vi "Start Sync.vi"(8 "error in (no error)":errorcluster, 11 "gRPC service in":refnum<class "OOBgRPCService.lvclass">) -> (0 "error out":errorcluster, 3 "gRPC service out":refnum<class "OOBgRPCService.lvclass">)   [LabVIEW 2025, in "OOB gRPC Server.lvlib" / "OOBgRPCService.lvclass"]
uses:
  OOBgRPCService.lvclass
  OOBgRPCService.lvclass/OOBgRPCService.ctl
  RPC Messages/hwval_GenericResponse.ctl
  <vilib>/xnet/xnet.llb/XNET Frame Type CAN.ctl
  RPC Messages/hwval_StatusResponse.ctl
  OOB Data Transfer/OOB Data Transfer.lvlib
  OOB gRPC Server.lvlib
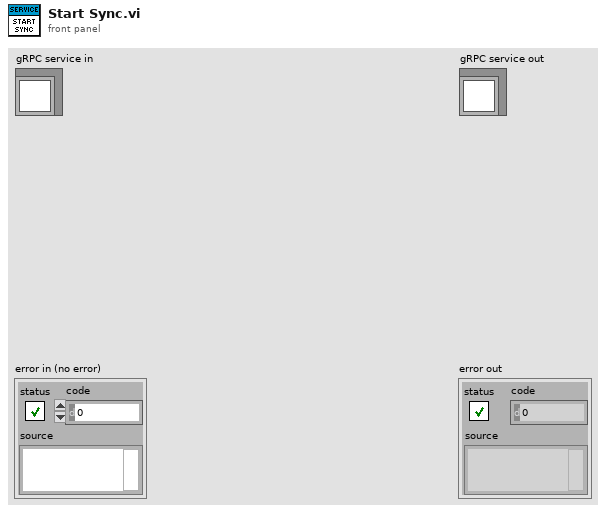
[diagram p1: front panel]
types:
  T1 = typedef "OOB gRPC Server.lvlib/hwval_GenericResponse.ctl" = cluster{"Payload":u8[]}
  T2 = typedef "OOB gRPC Server.lvlib/hwval_StatusResponse.ctl" = cluster{"Status":bool, "Code":i32, "Message":string}
  T3 = typedef "OOB gRPC Server.lvlib/OOBgRPCService.lvclass/Server Internal UEs.ctl" = cluster{"OOBgRPCService Generic Internal UE":refnum<user-event>, "OOBgRPCService PauseResume Internal UE":refnum<user-event>, "OOBgRPCService Export Internal UE":refnum<user-event>}
  T4 = typedef "OOB gRPC Server.lvlib/OOBgRPCService.lvclass/Server gRPC UEs.ctl" = cluster{"OOBgRPCService Generic gRPC UE":refnum<user-event>, "OOBgRPCService PauseResume gRPC UE":refnum<user-event>, "OOBgRPCService Export gRPC UE":refnum<user-event>}
  T5 = typedef "grpc-lvsupport-release.lvlib/grpcId.ctl" = u64
  T6 = typedef "OOB gRPC Server.lvlib/hwval_GenericRequest.ctl" = cluster{"Command":string, "Payload":u8[]}
  T7 = typedef "OOB Data Transfer.lvlib/OOB to Logic Data.ctl" = cluster{"PauseResume":bool, "Export":string, "ID CAN":u32, "Type CAN":T8, "DLC CAN":u32, "SEND CAN":bool, "Payload CAN":u32[], "ID LIN":u32, "DLC LIN":u32, "SEND LIN":bool, "Payload LIN":u32[], "out_str":string, "cfg err":bool}
  T8 = typedef "XNET Frame Type CAN.ctl" = u8
  T9 = typedef "OOB gRPC Server.lvlib/hwval_BoolRequest.ctl" = cluster{"BooleanData":bool}
  T10 = typedef "OOB gRPC Server.lvlib/hwval_ExportRequest.ctl" = cluster{"FileType":string}
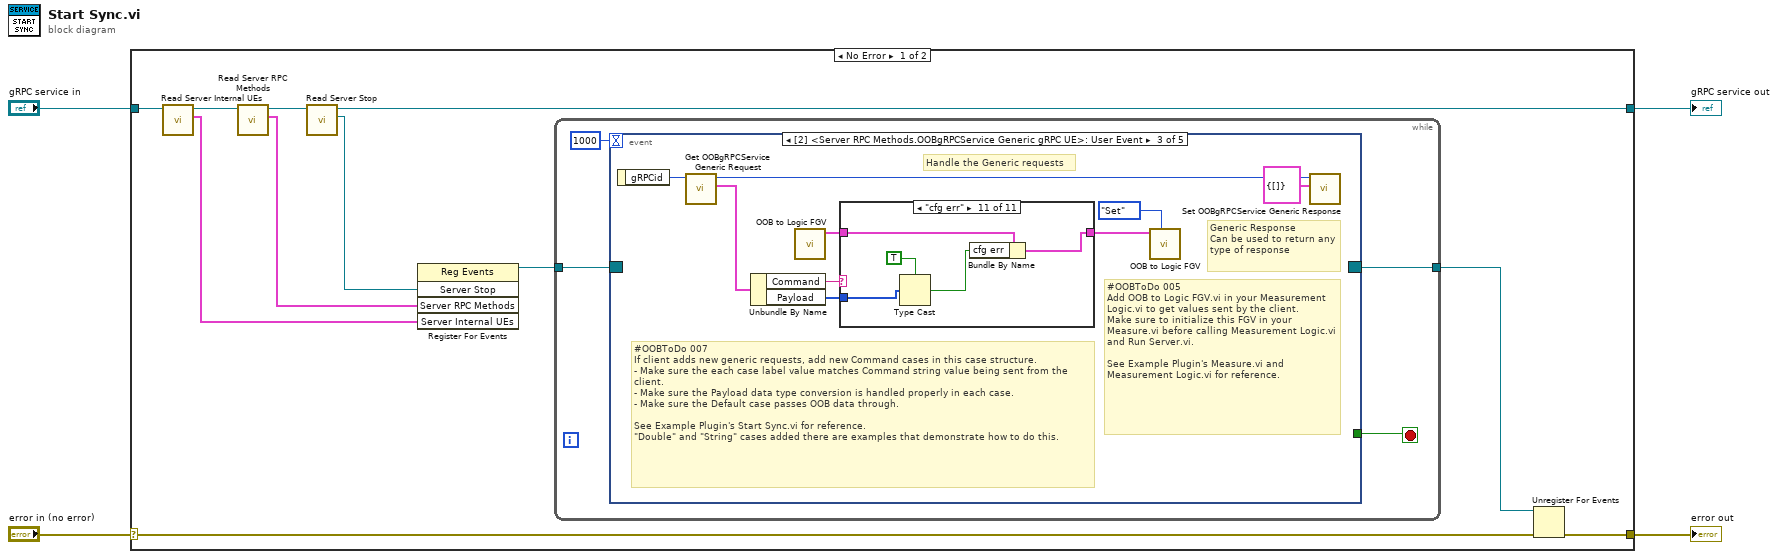
[diagram p0: block diagram]
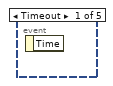
[diagram p2: hidden frame]
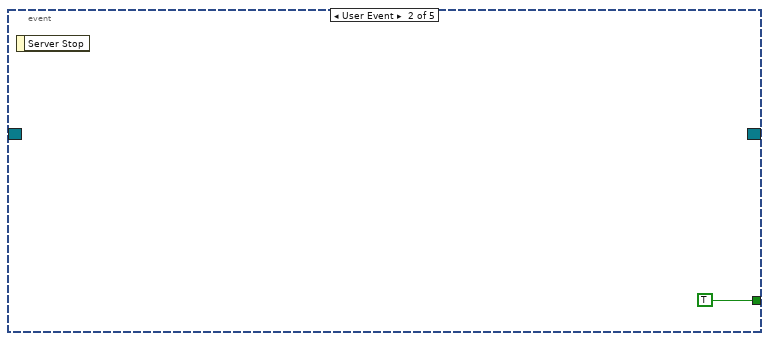
[diagram p3: hidden frame]
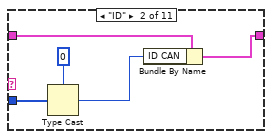
[diagram p5: hidden frame]
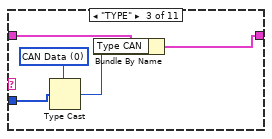
[diagram p6: hidden frame]
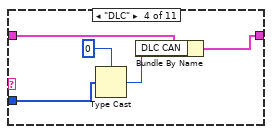
[diagram p7: hidden frame]
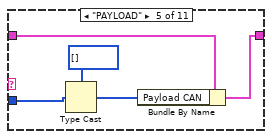
[diagram p8: hidden frame]
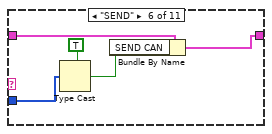
[diagram p9: hidden frame]
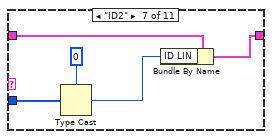
[diagram p10: hidden frame]
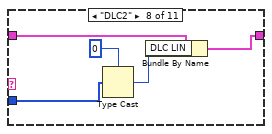
[diagram p11: hidden frame]
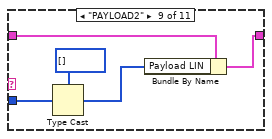
[diagram p12: hidden frame]
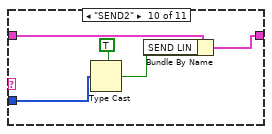
[diagram p13: hidden frame]
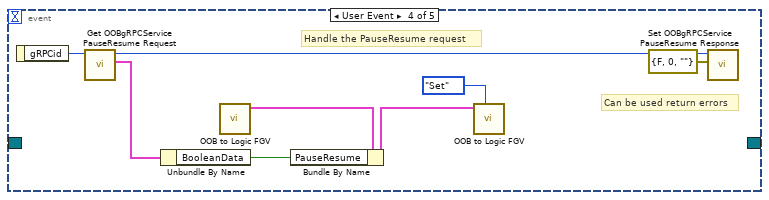
[diagram p14: hidden frame]
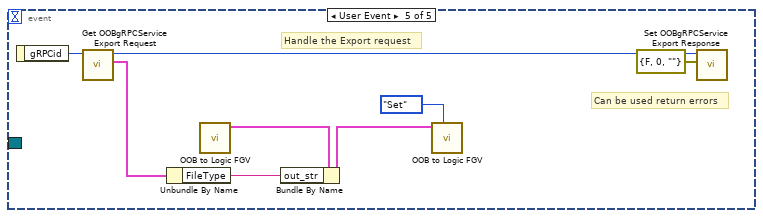
[diagram p15: hidden frame]
diagram:
  n1 = case shown="No Error" "error in (no error)" {
    selector: "error in (no error)" -> [w9 w98]
    tunnel: [w8 w98] -> w3
    tunnel: [w6 w97] -> w1
    tunnel: "gRPC service in" -> [w15 w97]
    frame No Error {
      n2 = call "Read Server Internal UEs.vi"("gRPC service in"=w15) -> ("Server Internal UEs"=w13:T3, "gRPC service out"=w14:refnum<class "OOBgRPCService.lvclass">)  [unwired: 8 in, 1 out]
      n3 = call "Read Server RPC Methods.vi"("gRPC service in"=w14) -> ("Server RPC Methods"=w7:T4, "gRPC service out"=w12:refnum<class "OOBgRPCService.lvclass">)  [unwired: 8 in, 1 out]
      n4 = call-dynamic "Read Server Stop.vi"("gRPC service in"=w12) -> ("Server Stop"=w5:refnum<user-event>, "gRPC service out"=w6:refnum<class "OOBgRPCService.lvclass">)  [unwired: 8 in, 1 out]
      n5 = register-events(w5, w7, w13) -> (reference out=w11:refnum<event-registration>)  [unwired: 2 in, 1 out]
      n6 = while {
        tunnel: w11 -> [w19]
        tunnel: [w17] -> w10
        stop <- w18 stop-if-true
        n7 = event "RPC Methods Event Structure" shown="[2] <Server RPC Methods.OOBgRPCService Generic gRPC UE>: User Event" {
          selector: w19 -> [_ _ _ _ _]
          dyn-events: [_ _ _ _ _] -> w17
          timeout: 1000 -> [_ _ _ _ _]
          tunnel: [_ TRUE _ _ _] -> w18
          event Timeout {
            n8 = event-data() -> ()  [unwired: 1 in, 1 out]
          }
          event User Event {
            n9 = event-data() -> ()  [unwired: 1 in, 1 out]
          }
          event User Event {
            # "#OOBToDo 007 \nIf client adds new generic requests, add new Command cases in this case structure. \n- Make sure the each case label value matches Command string value being sent from the client.\n- Make sure the Payload data type conversion is handled properly in each case.\n- Make sure the Default case passes OOB data through.\n\nSee Example Plugin's Start Sync.vi for reference. \n\"Double\" and \"String\" cases added there are examples that demonstrate how to do this."
            # "Handle the Generic requests"
            # "Generic Response\nCan be used to return any type of response"
            # "#OOBToDo 005 \nAdd OOB to Logic FGV.vi in your Measurement Logic.vi to get values sent by the client.\nMake sure to initialize this FGV in your Measure.vi before calling Measurement Logic.vi and Run Server.vi.\n\nSee Example Plugin's Measure.vi and Measurement Logic.vi for reference."
            n10 = event-data() -> ("gRPCid"=w29:T5)  [unwired: 1 in]
            n11 = call "Get OOBgRPCService Generic Request.vi"("gRPCid"=w29) -> ("Message Data"=w27:T6, "gRPCid out"=w28:T5)  [unwired: 8 in, 1 out]
            n12 = Unbundle By Name(w27) -> ("Command"=w22:string, "Payload"=w21:u8[])
            n13 = call "OOB to Logic FGV.vi"() -> ("OOB to Logic Data out"=w24:T7)  [unwired: 10 in, 1 out]
            n14 = case shown="\"cfg err\"" w22 {
              tunnel: w24 -> [w30 w35 w40 w45 w50 w55 w58 w62 w67 w71 w80]
              tunnel: [w30 w34 w39 w44 w49 w54 w57 w61 w66 w72 w79] -> w23
              tunnel: w21 -> [_ w33 w36 w41 w47 w51 w56 w63 w68 w73 w78]
              frame Default {
              }
              frame "ID" {
                n15 = Type Cast(type=u32 0 ("IDENTIFIER"), x=w33) -> (*(type *) &x=w31:u32)
                n16 = Bundle By Name(cluster=w35, "ID CAN"=w31) -> (w34:T7)
              }
              frame "TYPE" {
                w38 = T8 0 items=["CAN Data"=0, "CAN Remote"=1, "CAN Bus Error"=2, "CAN 2.0 Data"=8, "CAN FD Data"=16, "CAN FD+BRS Data"=24, "J1939 Data"=192, "Delay"=224, "Log Trigger"=225, "Start Trigger"=226] ("TYPE")
                n17 = Type Cast(type=w38, x=w36) -> (*(type *) &x=w37:T8)
                n18 = Bundle By Name(cluster=w40, "Type CAN"=w37) -> (w39:T7)
              }
              frame "DLC" {
                n19 = Type Cast(type=u32 0 ("DLC"), x=w41) -> (*(type *) &x=w42:u32)
                n20 = Bundle By Name(cluster=w45, "DLC CAN"=w42) -> (w44:T7)
              }
              frame "PAYLOAD" {
                n21 = Type Cast(type=u32[] [] ("PAYLOAD"), x=w47) -> (*(type *) &x=w46:u32[])
                n22 = Bundle By Name(cluster=w50, "Payload CAN"=w46) -> (w49:T7)
              }
              frame "SEND" {
                n23 = Type Cast(type=TRUE, x=w51) -> (*(type *) &x=w52:bool)
                n24 = Bundle By Name(cluster=w55, "SEND CAN"=w52) -> (w54:T7)
              }
              frame "ID2" {
                n25 = Type Cast(type=u32 0 ("IDENTIFIER"), x=w56) -> (*(type *) &x=w59:u32)
                n26 = Bundle By Name(cluster=w58, "ID LIN"=w59) -> (w57:T7)
              }
              frame "DLC2" {
                n27 = Type Cast(type=u32 0 ("DLC"), x=w63) -> (*(type *) &x=w64:u32)
                n28 = Bundle By Name(cluster=w62, "DLC LIN"=w64) -> (w61:T7)
              }
              frame "PAYLOAD2" {
                n29 = Type Cast(type=u32[] [] ("PAYLOAD"), x=w68) -> (*(type *) &x=w69:u32[])
                n30 = Bundle By Name(cluster=w67, "Payload LIN"=w69) -> (w66:T7)
              }
              frame "SEND2" {
                n31 = Type Cast(type=TRUE, x=w73) -> (*(type *) &x=w74:bool)
                n32 = Bundle By Name(cluster=w71, "SEND LIN"=w74) -> (w72:T7)
              }
              frame "cfg err" {
                n33 = Type Cast(type=TRUE, x=w78) -> (*(type *) &x=w76:bool)
                n34 = Bundle By Name(cluster=w80, "cfg err"=w76) -> (w79:T7)
              }
            }
            n35 = call "OOB to Logic FGV.vi"("Op (Get)"=enum16{"Get", "Set"}."Set", "OOB to Logic Data in"=w23) -> ()  [unwired: 8 in, 2 out]
            n36 = call "Set OOBgRPCService Generic Response.vi"("Message Data"=T1 {"Payload"=[]}, "gRPCid in"=w28) -> ()  [unwired: 9 in, 1 out]
          }
          event User Event {
            # "Handle the PauseResume request"
            # "Can be used return errors"
            n37 = event-data() -> ("gRPCid"=w82:T5)  [unwired: 1 in]
            n38 = call "Get OOBgRPCService PauseResume Request.vi"("gRPCid"=w82) -> ("Message Data"=w84:T9, "gRPCid out"=w85:T5)  [unwired: 8 in, 1 out]
            n39 = Unbundle By Name(w84) -> ("BooleanData"=w83:bool)
            n40 = call "OOB to Logic FGV.vi"() -> ("OOB to Logic Data out"=w87:T7)  [unwired: 10 in, 1 out]
            n41 = Bundle By Name(cluster=w87, "PauseResume"=w83) -> (w86:T7)
            n42 = call "OOB to Logic FGV.vi"("Op (Get)"=enum16{"Get", "Set"}."Set", "OOB to Logic Data in"=w86) -> ()  [unwired: 8 in, 2 out]
            n43 = call "Set OOBgRPCService PauseResume Response.vi"("Message Data"=T2 {"Status"=FALSE, "Code"=0, "Message"=""}, "gRPCid in"=w85) -> ()  [unwired: 9 in, 1 out]
          }
          event User Event {
            # "Handle the Export request"
            # "Can be used return errors"
            n44 = event-data() -> ("gRPCid"=w90:T5)  [unwired: 1 in]
            n45 = call "Get OOBgRPCService Export Request.vi"("gRPCid"=w90) -> ("Message Data"=w92:T10, "gRPCid out"=w96:T5)  [unwired: 8 in, 1 out]
            n46 = Unbundle By Name(w92) -> ("FileType"=w91:string)
            n47 = call "OOB to Logic FGV.vi"() -> ("OOB to Logic Data out"=w94:T7)  [unwired: 10 in, 1 out]
            n48 = Bundle By Name(cluster=w94, "out_str"=w91) -> (w93:T7)
            n49 = call "OOB to Logic FGV.vi"("Op (Get)"=enum16{"Get", "Set"}."Set", "OOB to Logic Data in"=w93) -> ()  [unwired: 8 in, 2 out]
            n50 = call "Set OOBgRPCService Export Response.vi"("Message Data"=T2 {"Status"=FALSE, "Code"=0, "Message"=""}, "gRPCid in"=w96) -> ()  [unwired: 9 in, 1 out]
          }
        }
      }
      n51 = Unregister For Events(event registration refnum=w10, error in=w9) -> (error out=w8:errorcluster)
    }
    frame Error {
    }
  }
  "error out" <- w3
  "gRPC service out" <- w1
